vi "Example - Write and Read Multiline Spreadsheet.vi"(8 "error in (no error)":errorcluster) -> (0 "error out":errorcluster)   [LabVIEW 2016, in "SLL Spreadsheet.lvlib"]
doc: "Example for Write Read Spreadsheet File with multi-line cell text."
uses:
  SLL Spreadsheet.lvlib
panel:
  out "Verified?":bool
  out "2D String[][] Out":string[][](array[string])
  in  "2D String[][]":string[][](array[string])=[["Normal Cell", "Cell with Multiple Lines", "Cell with quote in it "], ["My String", "Line 1\nLine 2\nLine 3", "He says: \"Hello World!\""], ["Item 1, Item 2", "", ""]]
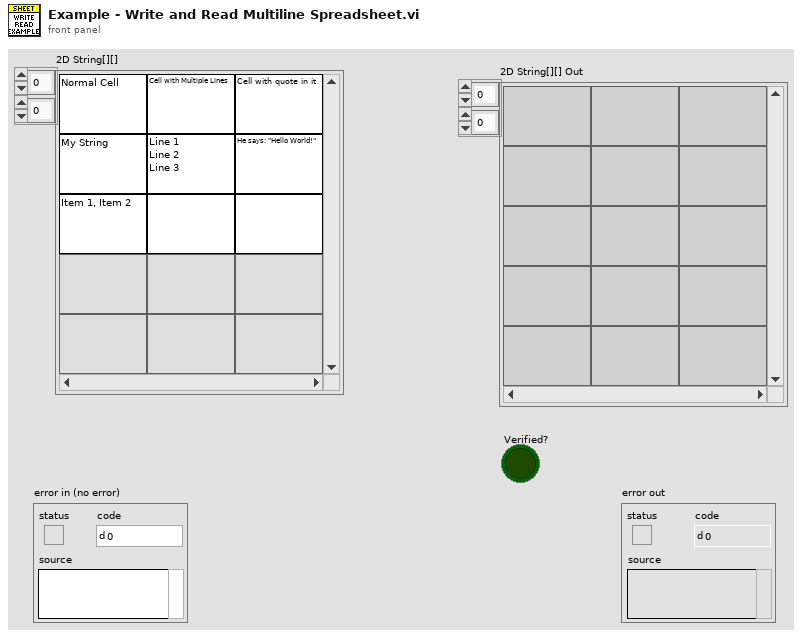
[diagram p1: front panel]
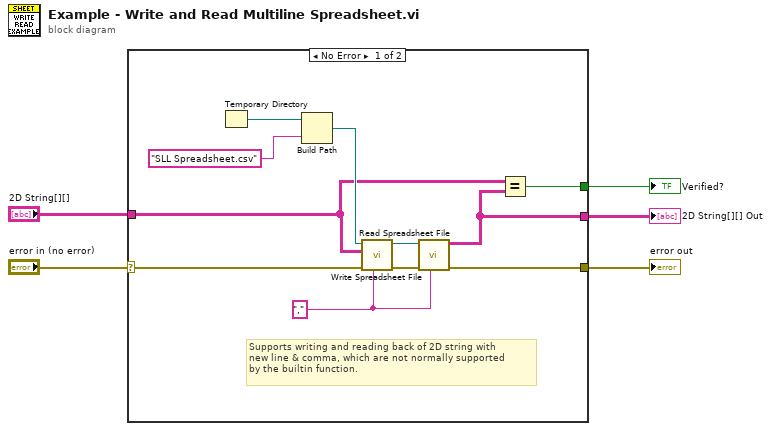
[diagram p0: block diagram]
diagram:
  n1 = case shown="No Error" "error in (no error)" {
    selector: "error in (no error)" -> [w14 w18]
    tunnel: [w9 w18] -> w4
    tunnel: [w8 w17] -> w3
    tunnel: "2D String[][]" -> [w7 w17]
    tunnel: [w6 _] -> w1
    frame No Error {
      w10 = "," ("Delimiter (tab)")
      # "Supports writing and reading back of 2D string with\nnew line & comma, which are not normally supported\nby the builtin function."
      n2 = Temporary Directory() -> (w16:path)
      n3 = Build Path(base path=w16, name or relative path="SLL Spreadsheet.csv") -> (appended path=w13:path)
      n4 = call "Write Spreadsheet File.vi"("Delimiter (tab)"=w10, "error in (no error)"=w14, "2D String[][]"=w7, "File Path"=w13) -> ("error out"=w12:errorcluster, "File Path dup"=w11:path)  [unwired: 6 in]
      n5 = call "Read Spreadsheet File.vi"("Delimiter (tab)"=w10, "error in (no error)"=w12, "File Path"=w11) -> ("error out"=w9:errorcluster, "2D Array"=w8:string[][])  [unwired: 7 in]
      n6 = Equal?(x=w7, y=w8) -> (x = y?=w6:bool)
    }
    frame Error {
    }
  }
  "error out" <- w4
  "2D String[][] Out" <- w3
  "Verified?" <- w1
